vi "lab3_1_rt.vi"() -> ()   [LabVIEW 2025]
uses:
  <vilib>/rvi/interface/nirviOpenFPGA/nirviOpenFPGA.xnode
  <vilib>/rvi/interface/nirviMethod/nirviMethod.xnode
  <vilib>/FPGAPlugInAG/Dynamic/niLvFpga_ConfigureFifo_Dynamic.vi
  <vilib>/rvi/errors/niLvFpgaMergeErrorWithErrorCode.vi
  <vilib>/rvi/interface/nirviReadWriteControl/nirviReadWriteControl.xnode
  NiFpgaLv.dll
  <vilib>/Utility/error.llb/Error Cluster From Error Code.vi
  <vilib>/rvi/interface/Simulation/niFpgaSimulationCallBeginRW.vi
  <vilib>/rvi/errors/niLvFpgaAdjustHostInterfaceError.vi
  <vilib>/FPGAPlugInAG/Dynamic/niLvFpga_Run_Dynamic.vi
  <vilib>/rvi/interface/nirviCloseFPGA/nirviCloseFPGA.xnode
  <vilib>/FPGAPlugInAG/Dynamic/niLvFpga_Close_Dynamic.vi
  <vilib>/FPGAPlugInAG/Dynamic/niLvFpga_ReadFifo_Dynamic.vi
panel:
  out "Elements Remaining":u32
  out "Waveform Graph":i16[](graph)
  out "error out":errorcluster
  in  "Treshold":i16
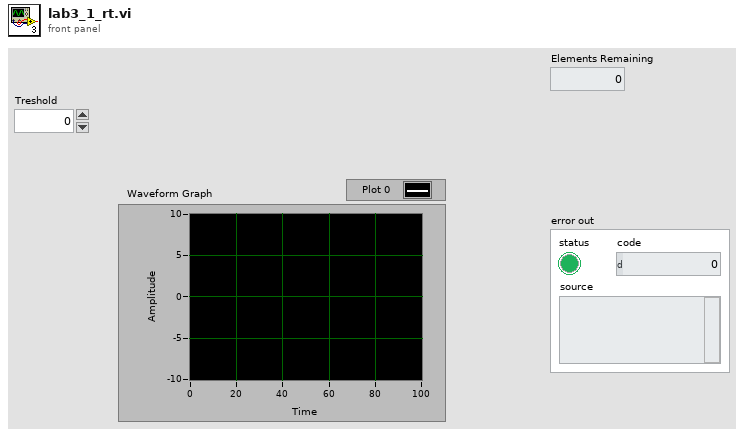
[diagram p1: front panel]
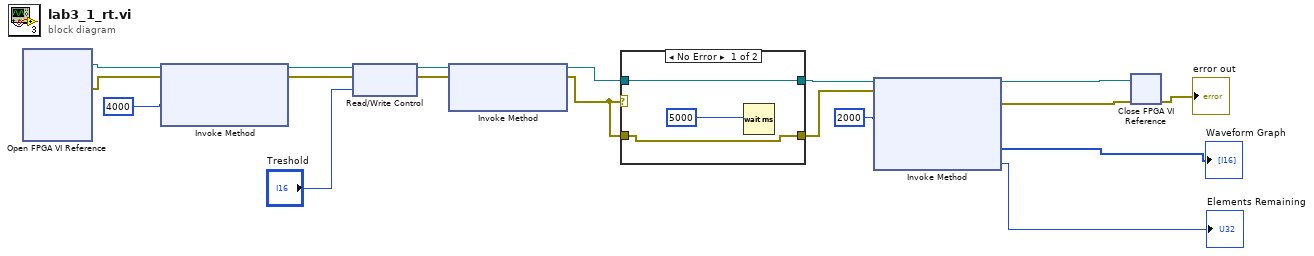
[diagram p0: block diagram]
diagram:
  n1 = xnode "Open FPGA VI Reference"() -> ("FPGA VI Reference Out"=w18:refnum<k20>, "error out"=w11:errorcluster)  [unwired: 2 in]
  n2 = xnode "Invoke Method"("FPGA VI Reference In"=w18, "error in"=w11, "Requested Depth"=u32 4000) -> ("FPGA VI Reference Out"=w16:refnum<k20>, "error out"=w12:errorcluster)  [unwired: 1 out]
  n3 = xnode "Read/Write Control"("FPGA VI Reference In"=w16, "error in"=w12, "Treshold"="Treshold") -> ("FPGA VI Reference Out"=w14:refnum<k20>, "error out"=w13:errorcluster)
  n4 = xnode "Invoke Method"("FPGA VI Reference In"=w14, "error in"=w13) -> ("FPGA VI Reference Out"=w7:refnum<k20>, "error out"=w5:errorcluster)  [unwired: 1 in]
  n5 = case shown="No Error" w5 {
    tunnel: w7 -> [w20 w23]
    tunnel: [w20 w23] -> w6
    tunnel: w5 -> [w19 w22]
    tunnel: [w19 w22] -> w4
    frame No Error {
      n6 = Wait (ms)(milliseconds to wait=u32 5000) -> ()  [unwired: 1 out]
    }
    frame Error {
    }
  }
  n7 = xnode "Invoke Method"("FPGA VI Reference In"=w6, "error in"=w4, "Number of Elements"=u32 2000) -> ("FPGA VI Reference Out"=w8:refnum<k20>, "error out"=w9:errorcluster, "Data"=→"Waveform Graph":i16[], "Elements Remaining"=→"Elements Remaining":u32)  [unwired: 1 in]
  n8 = xnode "Close FPGA VI Reference"("FPGA VI Reference In"=w8, "error in"=w9) -> ("error out"=→"error out":errorcluster)
